vi "Data Serie Calculation.vi"(9 "Operation":enum16{"A-B", "B-A", "A+B"}(ring), 10 "Data Serie B":T1, 11 "Data Serie A":T1) -> (2 "Waveform Out":waveform(dbl), 3 "Data Serie Out":T1)   [LabVIEW 2020, in "Data Viewer.lvlib" / "Data Viewer.lvclass"]
uses:
  Data Viewer.lvclass
  Data Serie--cluster.ctl
  <vilib>/measure/maresamp.llb/Resample Waveform (continuous).vi
  <vilib>/measure/NI_MAPro.lvlib
  Data Viewer.lvlib
panel:
  out "Waveform Chart":waveform(dbl)[](graph)
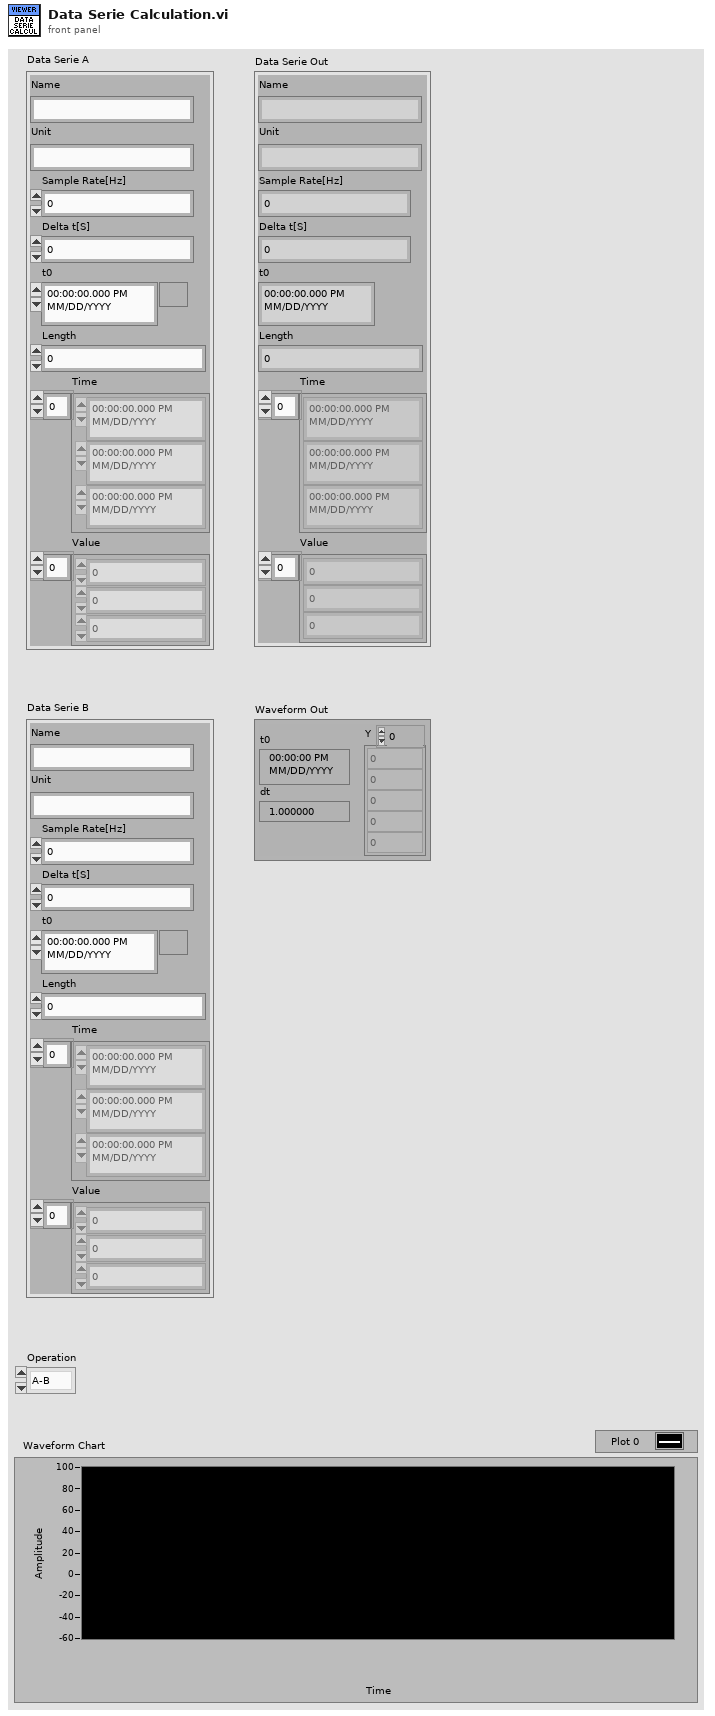
[diagram p1: front panel]
types:
  T1 = typedef "Data Viewer.lvlib/Data Serie--cluster.ctl" = cluster{"Name":string, "Unit":string, "Sample Rate[Hz]":dbl, "Delta t[S]":dbl, "t0":timestamp, "Length":i32, "Time":timestamp[], "Value":dbl[]}
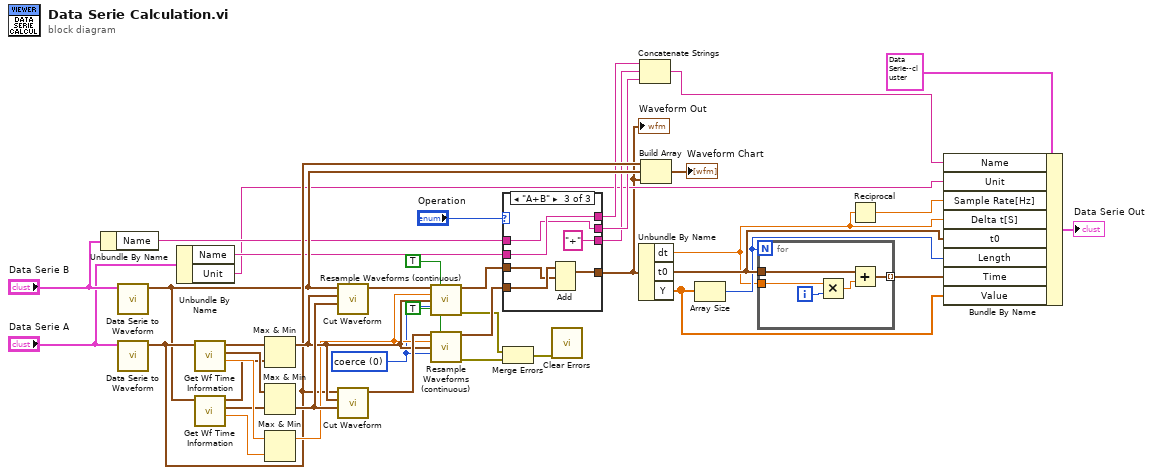
[diagram p0: block diagram]
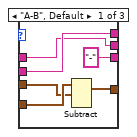
[diagram p2: hidden frame]
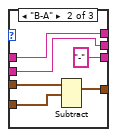
[diagram p3: hidden frame]
diagram:
  w9 = u16 0 items=["coerce", "linear", "spline", "FIR filter"] ("interpolation mode")
  n1 = Unbundle By Name("Data Serie B") -> ("Name"=w22:string)
  n2 = call "Data Serie to Waveform.vi"("Data Serie A"="Data Serie B") -> ("Waveform"=w28:waveform(dbl))  [unwired: 10 in]
  n3 = call "Data Serie to Waveform.vi"("Data Serie A"="Data Serie A") -> ("Waveform"=w29:waveform(dbl))  [unwired: 10 in]
  n4 = Unbundle By Name("Data Serie A") -> ("Name"=w23:string, "Unit"=w17:string)
  n5 = call "Get Wf Time Information.vi"("signal in"=w29) -> ("dt"=w39:dbl, "Final Time"=w40:timestamp, "Start Time"=w38:timestamp)  [unwired: 8 in]
  n6 = call "Get Wf Time Information.vi"("signal in"=w28) -> ("dt"=w35:dbl, "Final Time"=w36:timestamp, "Start Time"=w37:timestamp)  [unwired: 8 in]
  n7 = Max & Min(x=w38, y=w37) -> (max(x,y)=w31:timestamp)  [unwired: 1 out]
  n8 = Max & Min(x=w40, y=w36) -> (min(x,y)=w34:timestamp)  [unwired: 1 out]
  n9 = Max & Min(x=w39, y=w35) -> (max(x,y)=w30:dbl)  [unwired: 1 out]
  n10 = call "Cut Waveform.vi"("End Time"=w34, "Start Time"=w31, "Wafeform in"=w28) -> ("waveform out"=w32:waveform(dbl))  [unwired: 8 in]
  n11 = call "Cut Waveform.vi"("End Time"=w34, "Start Time"=w31, "Wafeform in"=w29) -> ("waveform out"=w33:waveform(dbl))  [unwired: 8 in]
  n12 = call-poly <vilib>:"Resample Waveforms (continuous).vi"("waveform in"=w32, "reset"=TRUE, "dt"=w30, "t0"=w31, "interpolation mode"=w9) -> ("resampled waveform out"=w25:waveform(dbl), "error out"=w8:errorcluster)  [unwired: 6 in, 3 out]
  n13 = call-poly <vilib>:"Resample Waveforms (continuous).vi"("waveform in"=w33, "reset"=TRUE, "dt"=w30, "t0"=w31, "interpolation mode"=w9) -> ("resampled waveform out"=w26:waveform(dbl), "error out"=w7:errorcluster)  [unwired: 6 in, 3 out]
  n14 = case shown="\"A+B\"" "Operation" {
    tunnel: w26 -> [w47 w52 w59]
    tunnel: w25 -> [w46 w53 w58]
    tunnel: [w45 w51 w57] -> w5
    tunnel: w23 -> [w44 w49 w56]
    tunnel: w22 -> [w43 w50 w55]
    tunnel: [w44 w50 w56] -> w21
    tunnel: [w43 w49 w55] -> w20
    tunnel: ["-" "-" "+"] -> w19
    frame "A-B", Default {
      n15 = Subtract(1:w46, 2:w47) -> (0:w45:waveform(dbl))  [unwired: 1 in, 1 out]
    }
    frame "B-A" {
      n16 = Subtract(1:w52, 2:w53) -> (0:w51:waveform(dbl))  [unwired: 1 in, 1 out]
    }
    frame "A+B" {
      n17 = Add(1:w58, 2:w59) -> (0:w57:waveform(dbl))  [unwired: 1 in, 1 out]
    }
  }
  "Waveform Out" <- w5
  n18 = Merge Errors(w8, w7) -> (w6:errorcluster)
  n19 = call <vilib>:"Clear Errors.vi"("error in (no error)"=w6) -> ()  [unwired: 5 in, 2 out]
  n20 = Unbundle By Name(w5) -> ("dt"=w12:dbl, "t0"=w14:timestamp, "Y"=w15:dbl[])
  n21 = Concatenate Strings(w21, w19, w20) -> (w18:string)
  n22 = Build Array(w29, w28, w5) -> (→"Waveform Chart":waveform(dbl)[])
  n23 = Array Size(array=w15) -> (size(s)=w13:i32)
  n24 = for {
    N: w13 -> [_]
    tunnel: w14 -> [w64]
    tunnel: w12 -> [w62]
    tunnel: [w60] -> w11 mode=indexing
    i -> [w63]
    n25 = Multiply(x=w62, y=w63) -> (x*y=w61:dbl)
    n26 = Add(x=w64, y=w61) -> (x+y=w60:timestamp)
  }
  n27 = Reciprocal(x=w12) -> (1/x=w16:dbl)
  n28 = Bundle By Name(cluster=T1 {"Name"="", "Unit"="", "Sample Rate[Hz]"=0.0, "Delta t[S]"=0.0, "t0"=timestamp(0 s since 1904-01-01), "Length"=0, "Time"=[], "Value"=[]} ("Data Serie B"), "Name"=w18, "Unit"=w17, "Sample Rate[Hz]"=w16, "Delta t[S]"=w12, "t0"=w14, "Length"=w13, "Time"=w11, "Value"=w15) -> (→"Data Serie Out":T1)
